vi "Get ControlRef from ClassItem.vi"(8 "error in (no error)":errorcluster, 10 "item name":string, 11 "class in":refnum<vi>) -> (0 "error out":errorcluster, 1 "found":bool, 2 "control":refnum<vi>, 3 "class out":refnum<vi>)   [LabVIEW 2019, in "gRPC Template Creation Utility.lvlib"]
uses:
  gRPC Template Creation Utility.lvlib
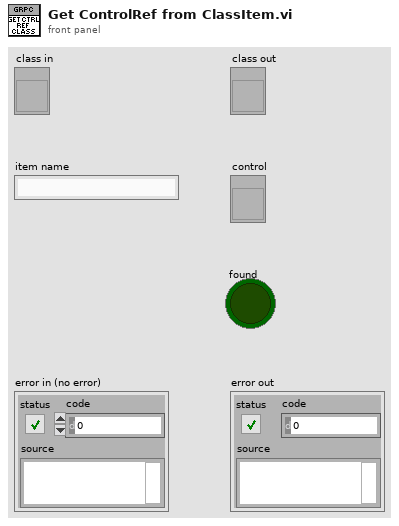
[diagram p1: front panel]
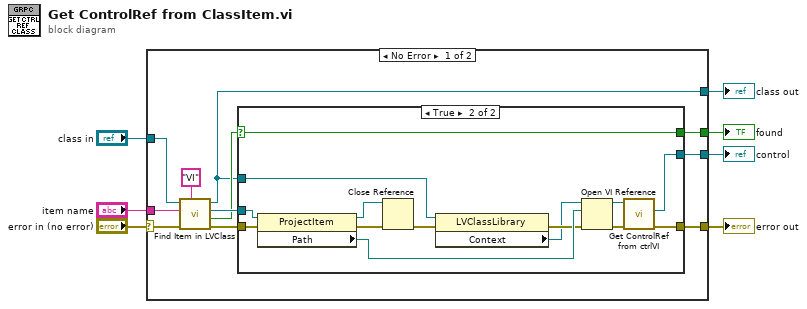
[diagram p0: block diagram]
diagram:
  n1 = case shown="No Error" "error in (no error)" {
    selector: "error in (no error)" -> [w11 w35]
    tunnel: [w18 _] -> w7
    tunnel: "class in" -> [w15 w36]
    tunnel: "item name" -> [w13 _]
    tunnel: [w8 w36] -> w4
    tunnel: [w12 w35] -> w3
    tunnel: [w9 _] -> w1
    frame No Error {
      n2 = call "Find Item in LVClass.vi"("Item Type"="VI", "error in (no error)"=w11, "Item Name"=w13, "Class Item in"=w15) -> ("error out"=w17:errorcluster, "Found?"=w10:bool, "Project Item (Class Item)"=w16:refnum<vi>, "Class Item out"=w8:refnum<vi>)  [unwired: 4 in]
      n3 = case shown="True" w10 {
        selector: w10 -> [w19 w28]
        tunnel: [_ w33] -> w18
        tunnel: w17 -> [w20 w31]
        tunnel: w16 -> [_ w30]
        tunnel: [w20 w21] -> w12
        tunnel: [w19 w28] -> w9
        tunnel: w8 -> [_ w27]
        frame False {
        }
        frame True {
          n4 = property class="ProjectItem"(reference=w30, error in=w31) -> (reference out=w22:refnum<vi>, error out=w24:errorcluster, "Path"=w29:path)
          n5 = Close Reference(reference=w22, error in (no error)=w24) -> (error out=w23:errorcluster)
          n6 = property class="LVClassLibrary"(reference=w27, error in=w23) -> (error out=w26:errorcluster, "Context"=w25:refnum<vi>)  [unwired: 1 out]
          n7 = Open VI Reference(application reference (local)=w25, vi path=w29, error in (no error)=w26) -> (vi reference=w32:refnum<vi>, error out=w34:errorcluster)  [unwired: 3 in]
          n8 = call "Get ControlRef from ctrlVI.vi"("error in (no error)"=w34, "VI ref in"=w32) -> ("error out"=w21:errorcluster, "Control ref out"=w33:refnum<vi>)  [unwired: 7 in, 1 out]
        }
      }
    }
    frame Error {
    }
  }
  "control" <- w7
  "class out" <- w4
  "error out" <- w3
  "found" <- w1
